vi "LHF.DB.Mongo.Collection.Core.Insert.vi"(8 "error in (no error)":errorcluster, 9 "collectionName":string, 10 "BsonDocument":refnum<k24>, 11 "LHF.DB.Mongo in":refnum<class "LHF.DB.Mongo.lvclass">) -> (0 "error out":errorcluster, 1 "Ok":bool, 2 "BsonDocument out":refnum<k24>, 3 "LHF.DB.Mongo out":refnum<class "LHF.DB.Mongo.lvclass">)   [LabVIEW 2013, in "LHF.DB.Mongo.lvclass"]
uses:
  LHF.DB.Mongo.lvclass
  C:/Users/Ricardo/Desktop/Projetos/LabVIEW-MongoDB/src/Driver/MongoDB.Bson.dll
  LabVIEW-MongoDB/src/Driver/MongoDB.Bson.dll
  C:/Users/Ricardo/Desktop/Projetos/LabVIEW-MongoDB/src/Driver/MongoDB.Driver.dll
  LabVIEW-MongoDB/src/Driver/MongoDB.Driver.dll
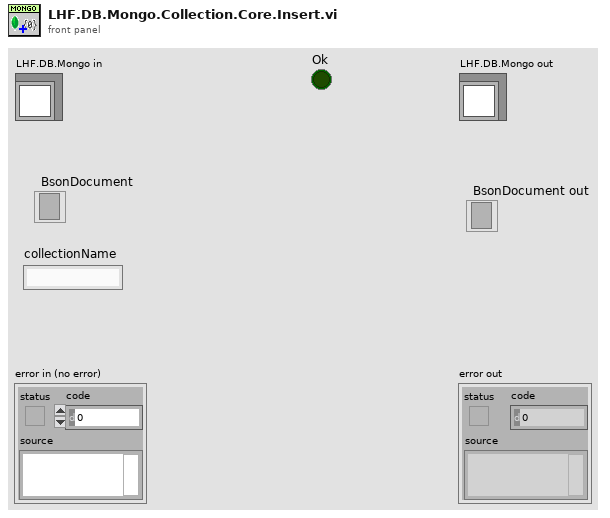
[diagram p1: front panel]
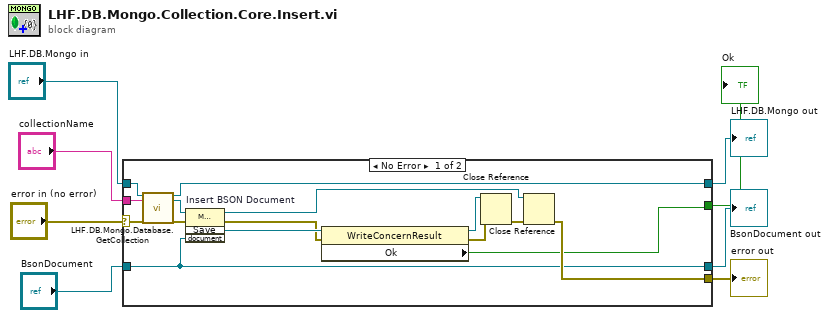
[diagram p0: block diagram]
diagram:
  n1 = case shown="No Error" "error in (no error)" {
    selector: "error in (no error)" -> [w22 w26]
    tunnel: [w16 w26] -> w7
    tunnel: [w18 w25] -> w5
    tunnel: "LHF.DB.Mongo in" -> [w19 w25]
    tunnel: "collectionName" -> [w23 _]
    tunnel: "BsonDocument" -> [w15 w24]
    tunnel: [w15 w24] -> w2
    tunnel: [w9 _] -> w1
    frame No Error {
      n2 = call "LHF.DB.Mongo.Database.GetCollection.vi"("LHF.DB.Mongo in"=w19, "collectionName"=w23, "error in (no error)"=w22) -> ("LHF.DB.Mongo in"=w18:refnum<class "LHF.DB.Mongo.lvclass">, "MongoCollection"=w21:refnum<k24>, "error out"=w20:errorcluster)  [unwired: 14 in]
      n3 = invoke on="Insert BSON Document" class="MongoCollection`1[[MongoDB.Bson" method="Save"(reference=w21, error in=w20, "document"=w15) -> (reference out=w17:refnum<k24>, error out=w11:errorcluster, "Save"=w14:refnum<k24>)  [unwired: 1 in, 1 out]
      n4 = property class="WriteConcernResult"(reference=w14, error in=w11) -> (reference out=w12:refnum<k24>, error out=w10:errorcluster, "Ok"=w9:bool)
      n5 = Close Reference(reference=w12, error in (no error)=w10) -> (error out=w13:errorcluster)
      n6 = Close Reference(reference=w17, error in (no error)=w13) -> (error out=w16:errorcluster)
    }
    frame Error {
    }
  }
  "error out" <- w7
  "LHF.DB.Mongo out" <- w5
  "BsonDocument out" <- w2
  "Ok" <- w1
